vi "Read Month.vi"(7 "Time Entry Store in":refnum<class "Time Entry Store.lvclass">, 8 "error in (no error)":errorcluster, 10 "Month":i32, 11 "Year":i32) -> (0 "error out":errorcluster, 3 "Time Entries":T1, 5 "Time Entry Store out":refnum<class "Time Entry Store.lvclass">)   [LabVIEW 2024, in "Time Entry Store.lvclass"]
doc: "Returns every time entry filed under the given month (by UTC Start Time), sorted by Start Time. The parent class has no storage: it returns empty results and does nothing. Time Entry Store-INI overrides it.\n\nGenerated by: Claude"
uses:
  Time Entry Store.lvclass
  Time Entry Store.lvclass/Time Entry Store.ctl
  Rows/Time Entry.ctl
  Rows/Time Entry List.ctl
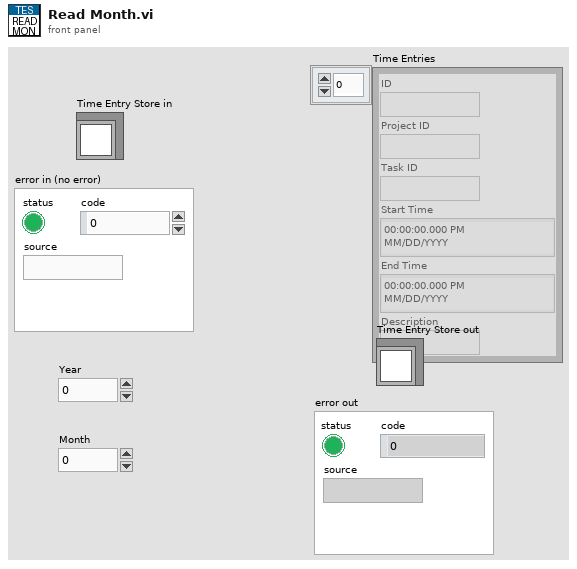
[diagram p1: front panel]
types:
  T1 = typedef "Time Entry List.ctl" = T2[]
  T2 = typedef "Time Entry.ctl" = cluster{"ID":string, "Project ID":string, "Task ID":string, "Start Time":timestamp, "End Time":timestamp, "Description":string}
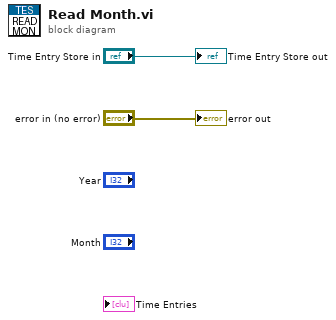
[diagram p0: block diagram]
diagram:
  "Time Entry Store out" <- "Time Entry Store in"
  "error out" <- "error in (no error)"
